vi "Highscore_Load.vi"(11 "error in":errorcluster) -> (4 "Table":cluster{"Score":i32, "Name":string}[](array[cluster]), 15 "error out":errorcluster)   [LabVIEW 2020, in "GH_Engine.lvlib"]
doc: "Reads the highscore list from Resourcesòta\\highscores.txt (one line per entry: Score;Name). Without the file or with an empty file the default list comes back and no error."
uses:
  GH_Engine.lvlib
  Level/GH_Level.lvlib
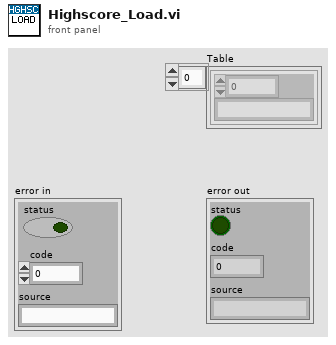
[diagram p1: front panel]
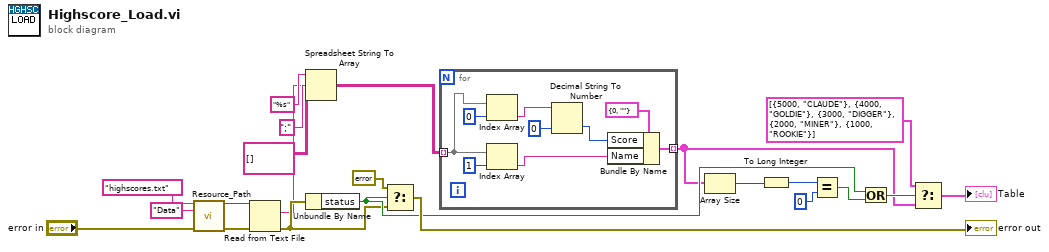
[diagram p0: block diagram]
diagram:
  n1 = call "Resource_Path.vi"("File name"="highscores.txt", "Subfolder"="Data", "error in"="error in") -> ("Path"=w4:path, "error out"=w5:errorcluster)  [unwired: 11 in]
  n2 = Read from Text File(file (use dialog)=w4, error in=w5) -> (text=w6:string, error out=w7:errorcluster)  [unwired: 2 in, 2 out]
  n3 = Spreadsheet String To Array(delimiter (Tab)=";", format string="%s", spreadsheet string=w6, array type (2D Dbl)=string[][] []) -> (array=w11:string[][])
  n4 = Unbundle By Name(w7) -> ("status"=w13:bool)
  n5 = Select(t=errorcluster {"status"=FALSE, "code"=0, "source"=""}, s=w13, f=w7) -> (s? t:f=→"error out":errorcluster)
  n6 = for {
    tunnel: w11 -> [w23] mode=indexing
    tunnel: [w31] -> w12 mode=indexing
    n7 = Index Array(array=w23, index=0) -> (element=w25:string)
    n8 = Index Array(array=w23, index=1) -> (element=w30:string)
    n9 = Decimal String To Number(string=w25, default (0L)=0) -> (number=w27:i32)  [unwired: 1 in, 1 out]
    n10 = Bundle By Name(cluster=cluster{"Score":i32, "Name":string} {"Score"=0, "Name"=""}, "Score"=w27, "Name"=w30) -> (w31:cluster{"Score":i32, "Name":string})
  }
  n11 = Array Size(array=w12) -> (size(s)=w14:i32)
  n12 = To Long Integer(number=w14) -> (32bit integer=w15:i32)
  n13 = Equal?(x=w15, y=0) -> (x = y?=w17:bool)
  n14 = Or(x=w13, y=w17) -> (x .or. y?=w18:bool)
  n15 = Select(t=cluster{"Score":i32, "Name":string}[] [{"Score"=5000, "Name"="CLAUDE"}, {"Score"=4000, "Name"="GOLDIE"}, {"Score"=3000, "Name"="DIGGER"}, {"Score"=2000, "Name"="MINER"}, {"Score"=1000, "Name"="ROOKIE"}] ("Default list"), s=w18, f=w12) -> (s? t:f=→"Table":cluster{"Score":i32, "Name":string}[])
